vi "Orange--constant.vi"() -> (1 "Orange":u32(colorbox))   [LabVIEW 2018, in "Band Colors.lvlib"]
doc: "Provides the RGB color value for orange.\n\nThe VI converts the RGB components (255, 128, 0) into a LabVIEW color value and returns it through <b>Orange</b>."
uses:
  Band Colors.lvlib
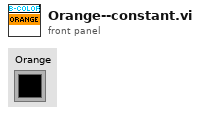
[diagram p1: front panel]
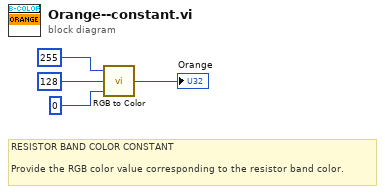
[diagram p0: block diagram]
diagram:
  # "RESISTOR BAND COLOR CONSTANT\n\nProvide the RGB color value corresponding to the resistor band color."
  n1 = call <vilib>:"RGB to Color.vi"("B"=u8 0, "G"=u8 128, "R"=u8 255) -> ("Color"=→"Orange":u32)
